vi "cal.vi"() -> ()   [LabVIEW 2018]
panel:
  out "?":dbl(graph)
  in  "Control":string
  in  "NUM_2":dbl
  out "OUTPUT":dbl
  in  "NUM_1":dbl
  # "CALCULATOR(--> +,-,*./,NOR)"
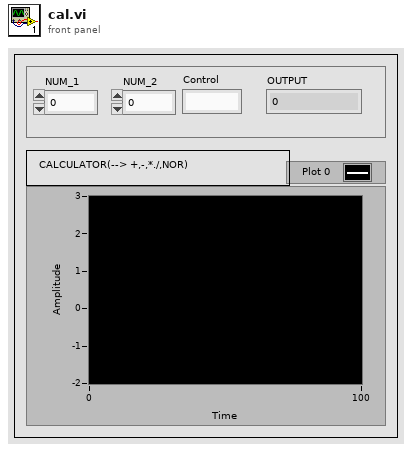
[diagram p1: front panel]
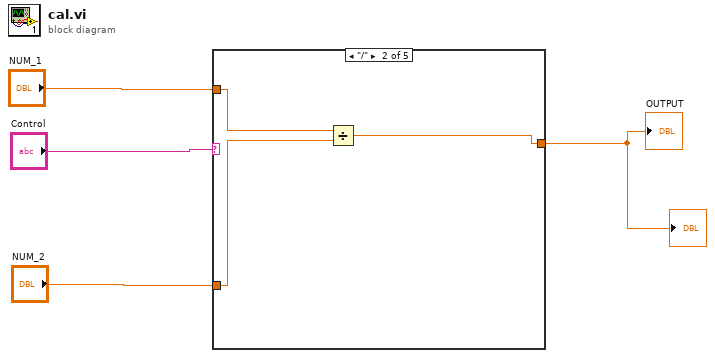
[diagram p0: block diagram]
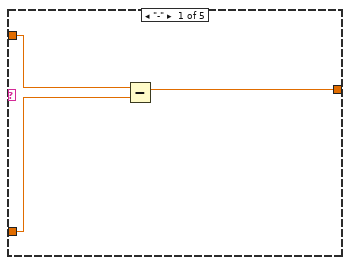
[diagram p2: hidden frame]
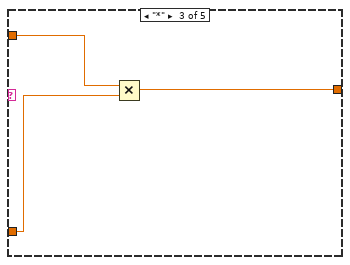
[diagram p3: hidden frame]
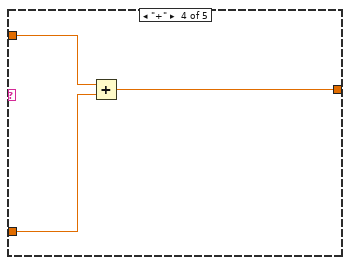
[diagram p4: hidden frame]
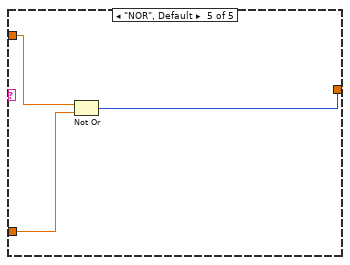
[diagram p5: hidden frame]
diagram:
  n1 = case shown="\"/\"" "Control" {
    tunnel: "NUM_1" -> [w6 w10 w13 w16 w19]
    tunnel: "NUM_2" -> [w5 w9 w12 w15 w18]
    tunnel: [w7 w8 w11 w14 w17] -> w1
    frame "-" {
      n2 = Subtract(x=w6, y=w5) -> (x-y=w7:dbl)
    }
    frame "/" {
      n3 = Divide(x=w10, y=w9) -> (x/y=w8:dbl)
    }
    frame "*" {
      n4 = Multiply(x=w13, y=w12) -> (x*y=w11:dbl)
    }
    frame "+" {
      n5 = Add(x=w16, y=w15) -> (x+y=w14:dbl)
    }
    frame "NOR", Default {
      n6 = Not Or(1:w18, 2:w19) -> (0:w17:i32)
    }
  }
  "OUTPUT" <- w1
  "?" <- w1
